vi "UnInstallGRPCPackages.vi"(7 "labview version":string, 8 "error in":errorcluster) -> (0 "error out":errorcluster)   [LabVIEW 2019]
uses:
  <vilib>/JKI/VIPM API/VIPM API_vipm_api.lvlib
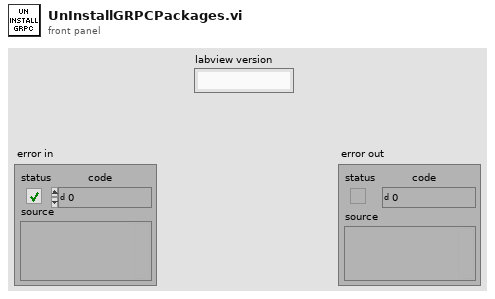
[diagram p1: front panel]
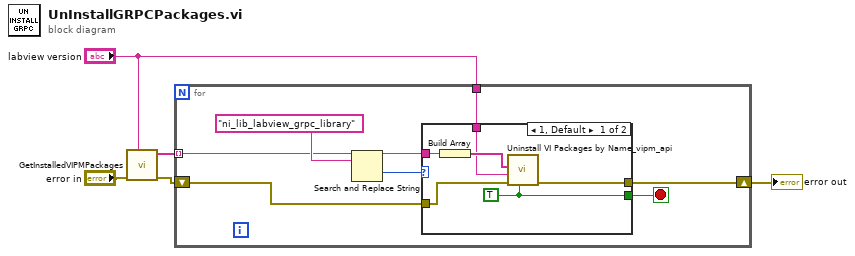
[diagram p0: block diagram]
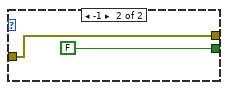
[diagram p2: hidden frame]
diagram:
  n1 = call "GetInstalledVIPMPackages.vi"("labview version"="labview version", "error in"="error in") -> ("error out"=w2:errorcluster, "array"=w5:string[])  [unwired: 8 in]
  n2 = for {
    tunnel: w5 -> [w9] mode=indexing
    tunnel: "labview version" -> [w8]
    shift-right: [w6] -> w1
    shift-left: w2 -> [w7]
    stop <- w10 stop-if-true
    n3 = Search and Replace String(input string=w9, search string="ni_lib_labview_grpc_library") -> (offset past replacement=w11:i32)  [unwired: 6 in, 3 out]
    n4 = case shown="1, Default" w11 {
      tunnel: [w18 FALSE ("quiet? (T)")] -> w10
      tunnel: w9 -> [w17 _]
      tunnel: w8 -> [w15 _]
      tunnel: w7 -> [w14 w19]
      tunnel: [w13 w19] -> w6
      frame 1, Default {
        w18 = TRUE ("quiet? (T)")
        n5 = Build Array(w17) -> (w16:string[])
        n6 = call <vilib>:"Uninstall VI Packages by Name_vipm_api.vi"("quiet? (T)"=w18, "error in (no error)"=w14, "LabVIEW Version"=w15, "Package Names to Uninstall []"=w16) -> ("error out"=w13:errorcluster)  [unwired: 7 in]
      }
      frame -1 {
      }
    }
  }
  "error out" <- w1
